vi "MultiProcess.vi"(0 "VI Reference In":refnum<vi>, 2 "Label":string, 5 "Wash Array":T1[](array[typedef])=[{"Wash Option"="Underbody Wash", "Car Position"=1, "Elapsed Time"=5.0}, {"Wash Option"="Bug Remover", "Car Position"=1, "Elapsed Time"=5.0}, {"Wash Option"="Pre-Soak", "Car Position"=2, "Elapsed Time"=2.0}, {"Wash Option"="High Pressure Wash", "Car Position"=2, "Elapsed Time"=5.0}, {"Wash Option"="Low Pressure Wax", "Car Position"=2, "Elapsed Time"=5.0}, {"Wash Option"="Spot Free Rinse", "Car Position"=2, "Elapsed Time"=5.0}, {"Wash Option"="Tire Shine Foam", "Car Position"=3, "Elapsed Time"=5.0}, {"Wash Option"="Air Dry", "Car Position"=3, "Elapsed Time"=5.0}], 11 "error in":errorcluster) -> (4 "VI Reference Out":refnum<vi>, 15 "error out":errorcluster)   [LabVIEW 2016, in "CarWashTest.lvlib"]
doc: "Multi process test"
uses:
  CarWashTest.lvlib
  Controls/WashStepConfig.ctl
  APIs/Stimulus/ControlValue/ValueSignalByPathString.vi
  APIs/Stimulus/ControlValue/ValueSignalLatchBooleanString.vi
  APIs/Assert/AssertControlProperty/AssertControlDisable/AssertDisabledAndGrayedOut.vi
  APIs/Assert/AssertControlValue/True.vi
  APIs/Stimulus/ControlValue/SetValueAuto.vi
  Drona.lvlib
  <vilib>/addons/_JKI Toolkits/Caraya/classes/Test/Test.lvclass
  APIs/Assert/AssertControlValue/AssertControlValue.lvlib
  APIs/Assert/AssertControlProperty/AssertControlDisable/AssertControlDisable.lvlib
  APIs/Stimulus/ControlValue/ControlValue.lvlib
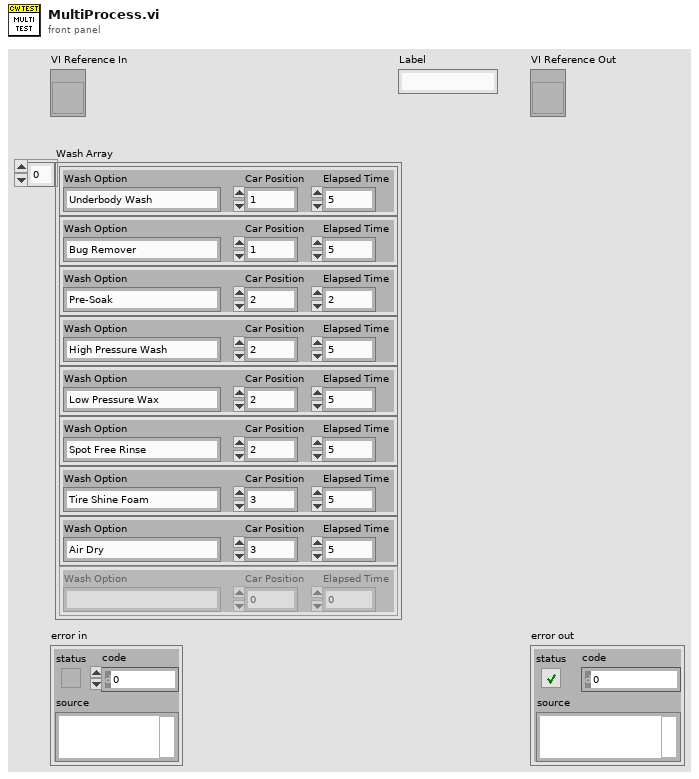
[diagram p1: front panel]
types:
  T1 = typedef "CarWashTest.lvlib/WashStepConfig.ctl" = cluster{"Wash Option":string, "Car Position":i32, "Elapsed Time":dbl}
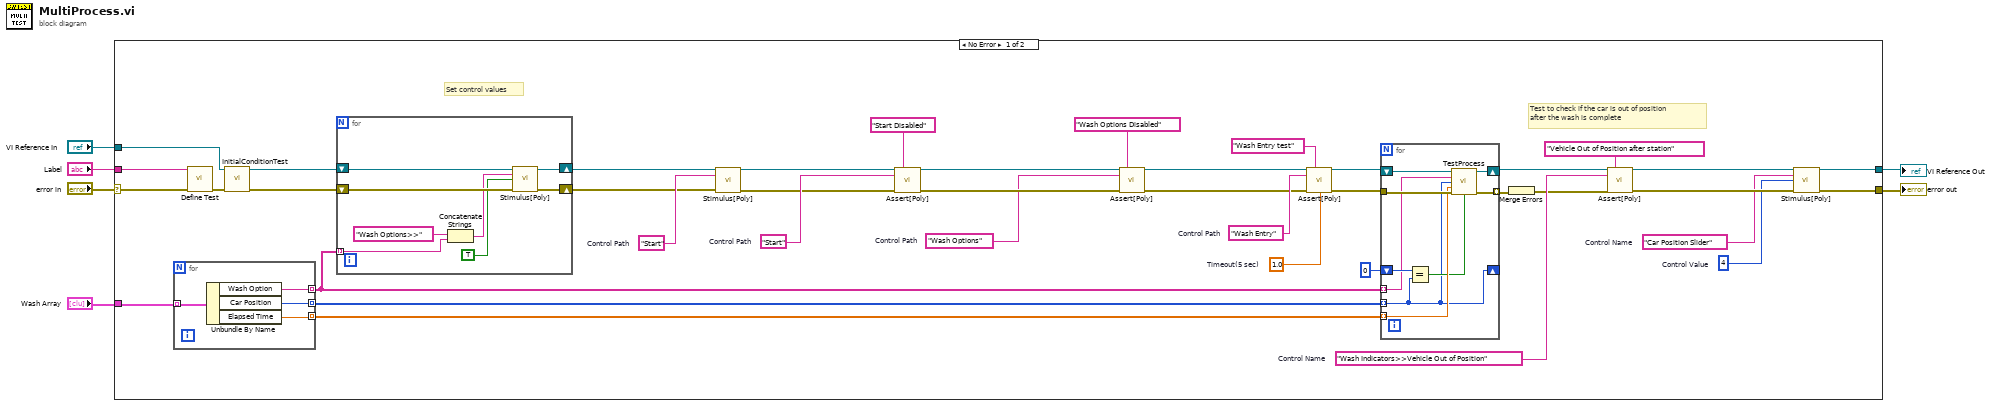
[diagram p0: block diagram]
diagram:
  n1 = case shown="No Error" "error in" {
    selector: "error in" -> [w35 w69]
    tunnel: "VI Reference In" -> [w45 w68]
    tunnel: [w42 w68] -> w5
    tunnel: [w41 w69] -> w4
    tunnel: "Label" -> [w40 _]
    tunnel: "Wash Array" -> [w17 _]
    frame No Error {
      w12 = "Start"  # Control Path
      w14 = "Wash Options"  # Control Path
      w39 = "Start"  # Control Path
      w32 = 4  # Control Value
      w31 = "Car Position Slider"  # Control Name
      w29 = "Wash Indicators>>Vehicle Out of Position"  # Control Name
      w28 = 1.0  # Timeout(5 sec)
      w27 = "Wash Entry"  # Control Path
      # "Set control values"
      # "Test to check if the car is out of position \nafter the wash is complete"
      n2 = for {
        tunnel: w17 -> [w50] mode=indexing
        tunnel: [w49] -> w20 mode=indexing
        tunnel: [w48] -> w22 mode=indexing
        tunnel: [w47] -> w21 mode=indexing
        n3 = Unbundle By Name(w50) -> ("Wash Option"=w49:string, "Car Position"=w48:i32, "Elapsed Time"=w47:dbl)
      }
      n4 = call <vilib>:"Define Test.vi"("error in (no error)"=w35, "Label (VI Title)"=w40) -> ("error out"=w43:errorcluster)  [unwired: 8 in, 1 out]
      n5 = call "InitialConditionTest.vi"("VI Reference In"=w45, "error in"=w43) -> ("VI Reference Out"=w46:refnum<vi>, "error out"=w44:errorcluster)  [unwired: 12 in]
      n6 = for {
        tunnel: w20 -> [w56] mode=indexing
        shift-right: [w55] -> w37
        shift-left: w46 -> [w58]
        shift-right: [w54] -> w36
        shift-left: w44 -> [w57]
        n7 = Concatenate Strings("Wash Options>>", w56) -> (w52:string)
        n8 = call-poly "Stimulus[Poly].vi"("VI Reference In"=w58, "Control Path"=w52, "Value (Signaling)"=TRUE, "error in"=w57) -> ("VI Reference Out"=w55:refnum<vi>, "error out"=w54:errorcluster)  [unwired: 10 in]
      }
      n9 = call-poly "Stimulus[Poly].vi"("VI Reference In"=w37, "Control Path"=w39, "error in"=w36) -> ("VI Reference Out"=w10:refnum<vi>, "error out"=w8:errorcluster)  [unwired: 11 in]
      n10 = call-poly "Assert[Poly].vi"("VI Reference In"=w10, "Test Label"="Start Disabled", "Control Path"=w12, "Error In"=w8) -> ("VI Reference Out"=w13:refnum<vi>, "Error Out"=w15:errorcluster)  [unwired: 9 in, 1 out]
      n11 = call-poly "Assert[Poly].vi"("VI Reference In"=w13, "Test Label"="Wash Options Disabled", "Control Path"=w14, "Error In"=w15) -> ("VI Reference Out"=w9:refnum<vi>, "Error Out"=w7:errorcluster)  [unwired: 9 in, 1 out]
      n12 = call-poly "Assert[Poly].vi"("VI Reference In"=w9, "Test Label"="Wash Entry test" ("Label"), "Control Path"=w27, "Error In"=w7, "Timeout(5 sec)"=w28) -> ("VI Reference Out"=w23:refnum<vi>, "Error Out"=w24:errorcluster)  [unwired: 8 in, 1 out]
      n13 = for {
        tunnel: w22 -> [w60] mode=indexing
        tunnel: w21 -> [w64] mode=indexing
        shift-right: [w62] -> w19
        shift-left: w23 -> [w65]
        shift-right: [w60] -> _
        shift-left: u8 0 ("Car Position") -> [w67]
        tunnel: w20 -> [w59] mode=indexing
        tunnel: w24 -> [w66]
        tunnel: [w61] -> w18 mode=indexing
        n14 = Equal?(x=w67, y=w60) -> (x = y?=w63:bool)
        n15 = call "TestProcess.vi"("VI Reference In"=w65, "Wash Option"=w59, "Car Position"=w60, "Elapsed Time"=w64, "error in"=w66, "Same Position?"=w63) -> ("VI Reference Out"=w62:refnum<vi>, "error out"=w61:errorcluster)  [unwired: 8 in]
      }
      n16 = Merge Errors(w18) -> (w26:errorcluster)
      n17 = call-poly "Assert[Poly].vi"("VI Reference In"=w19, "Test Label"="Vehicle Out of Position after station" ("Label"), "Control Path"=w29, "Error In"=w26) -> ("VI Reference Out"=w33:refnum<vi>, "Error Out"=w34:errorcluster)  [unwired: 9 in, 1 out]
      n18 = call-poly "Stimulus[Poly].vi"("VI Reference In"=w33, "Control Path"=w31, "Value (Signaling)"=w32, "error in"=w34) -> ("VI Reference Out"=w42:refnum<vi>, "error out"=w41:errorcluster)  [unwired: 10 in]
    }
    frame Error {
    }
  }
  "error out" <- w4
  "VI Reference Out" <- w5
